vi "read_Array.vi"(8 "错误输入（无错误）":errorcluster, 10 "Address":string, 11 "URL":string="opc://localhost/National Instruments.NIOPCServers.V5/Channel1.Battery_Testing.") -> (0 "error out":errorcluster caption="错误输出", 2 "Value":u8[](array[numeric]), 3 "ok?":bool)   [LabVIEW 2013]
panel:
  out "数据":u16
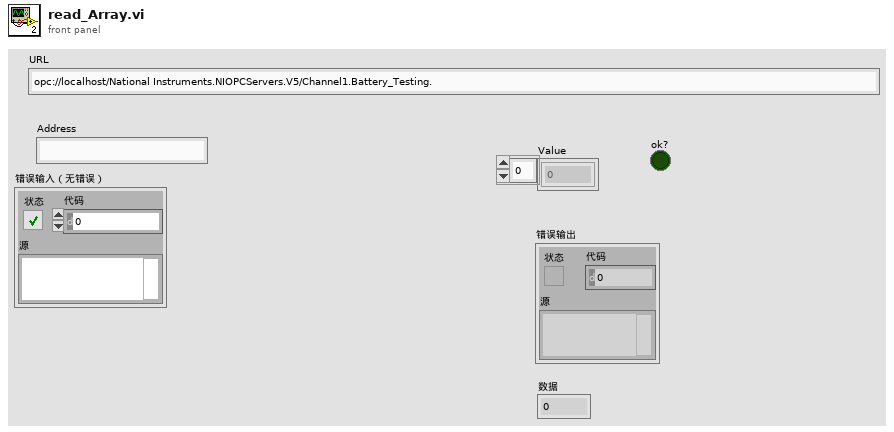
[diagram p1: front panel]
types:
  T1 = enum16{"Read", "Write", "ReadWrite", "BufferedRead", "BufferedReadWrite"}
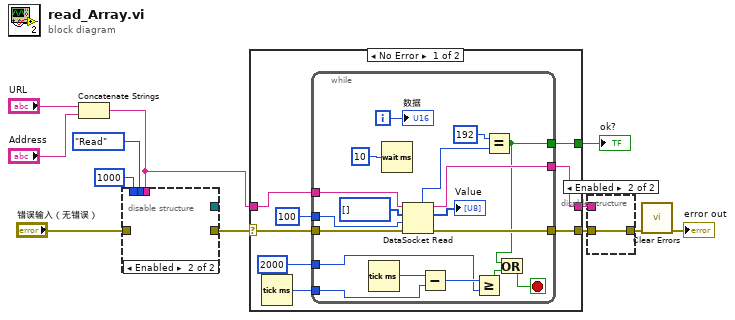
[diagram p0: block diagram]
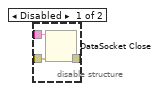
[diagram p2: hidden frame]
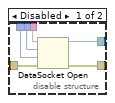
[diagram p3: hidden frame]
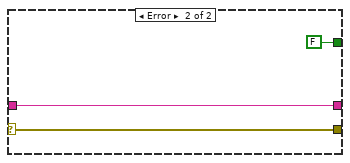
[diagram p4: hidden frame]
diagram:
  n1 = Concatenate Strings("URL", "Address") -> (w1:string)
  n2 = disable-structure shown="Enabled" {
    disable-tunnel: w1 -> [w18 _]
    disable-tunnel: T1."Read" ("模式") -> [w17 _]
    disable-tunnel: 1000 ("毫秒超时(10000)") -> [w16 _]
    disable-tunnel: [w15 _] -> _
    disable-tunnel: [w14 _] -> w4
    disable-tunnel: "错误输入（无错误）" -> [w13 _]
    frame Disabled {
      n3 = DataSocket Open(8:w13, 9:w16, 10:w17, 11:w18) -> (0:w14:errorcluster, 3:w15:refnum<k13>)
    }
    frame Enabled {
    }
  }
  n4 = case shown="No Error" w4 {
    selector: w4 -> [w22 w45]
    tunnel: w1 -> [w25 w47]
    tunnel: [w24 w47] -> w8
    tunnel: [w23 w45] -> w7
    tunnel: [w21 FALSE ("timed out")] -> w3
    frame No Error {
      n5 = Tick Count (ms)() -> (millisecond timer value=w19:u32)
      n6 = while {
        tunnel: 100 ("毫秒超时(0)") -> [w43]
        tunnel: w22 -> [w42]
        tunnel: w25 -> [w41]
        tunnel: [w40] -> w24
        tunnel: [w39] -> w23
        tunnel: [w28] -> w21
        tunnel: 2000 ("毫秒超时(0)") -> [w30]
        tunnel: w19 -> [w32]
        i -> [w38]
        stop <- w27 stop-if-true
        n7 = Tick Count (ms)() -> (millisecond timer value=w33:u32)
        n8 = Wait (ms)(milliseconds to wait=u32 10 ("等待时间（毫秒）")) -> ()  [unwired: 1 out]
        n9 = DataSocket Read(8:w42, 9:w43, 10:u8[] [] ("Value"), 11:w41) -> (0:w39:errorcluster, 2:→"Value":u8[], 3:w40:string, 5:w37:u64)  [unwired: 1 in, 3 out]
        n10 = Subtract(x=w33, y=w32) -> (x-y=w31:u32)
        n11 = Greater Or Equal?(x=w31, y=w30) -> (x >= y?=w29:bool)
        n12 = Equal?(x=u64 192, y=w37) -> (x = y?=w28:bool)
        n13 = Or(x=w28, y=w29) -> (x .or. y?=w27:bool)
        "数据" <- w38
      }
    }
    frame Error {
    }
  }
  "ok?" <- w3
  n14 = disable-structure shown="Enabled" {
    disable-tunnel: w8 -> [w50 _]
    disable-tunnel: w7 -> [w49 w51]
    disable-tunnel: [w48 w51] -> w6
    frame Disabled {
      n15 = DataSocket Close(8:w49, 11:w50) -> (0:w48:errorcluster)  [unwired: 1 in, 1 out]
    }
    frame Enabled {
    }
  }
  n16 = call <vilib>:"Clear Errors.vi"("error in (no error)"=w6) -> ("error out"=→"error out":errorcluster)  [unwired: 6 in]
